vi "Initialization.vi"(8 "error in":errorcluster, 9 "UI Refs":T1, 10 "user event":T2, 11 "XY Plotter":refnum<class "XY Plotter.lvclass">) -> (0 "error out":errorcluster, 3 "XY Plotter out":refnum<class "XY Plotter.lvclass">)   [LabVIEW 2025, in "XY Plotter.lvlib" / "XY Plotter.lvclass"]
uses:
  XY Plotter.lvclass
  Users/Public/Documents/Sandia National Labs/TSS Plugin/CEF.lvlibp/Node/UserEventRef.ctl
  XY Plotter.lvclass/XY Plotter.ctl
  XY Plotter configuration/XY Plotter configuration.lvclass/XY Plotter configuration.ctl
  XY Plotter configuration/Read XY Plotter.vi
  XY Plotter configuration/XY Plotter configuration.lvclass
  Users/Public/Documents/Sandia National Labs/TSS Plugin/CEF.lvlibp/Node/CEF_Node.lvclass
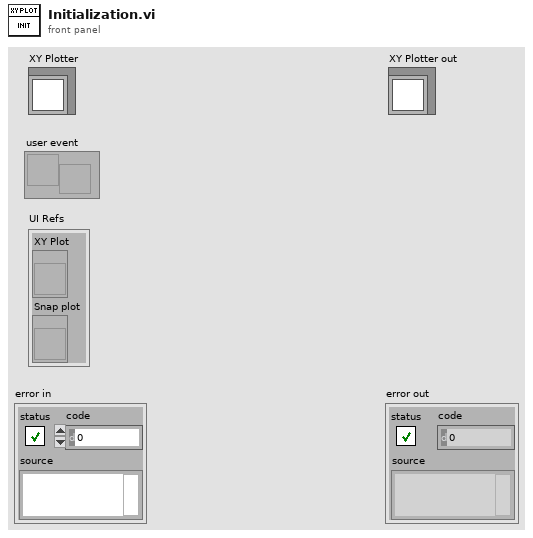
[diagram p1: front panel]
types:
  T1 = cluster{"XY Plot":refnum<vi>, "Snap plot":refnum<vi>}
  T2 = typedef "CEF.lvlibp/CEF_Node.lvclass/UserEventRef.ctl" = refnum<user-event>
  T3 = typedef "XY Plotter.lvlib/XY Plotter configuration.lvclass/XY Plotter.ctl" = cluster{"Data Rate":i32, "Y-Scales":cluster{"Label":string, "Max":dbl, "Min":dbl, "Unit":enum16{"---", "V", "mA", "sec", "dB", "deg", "in/s", "in", "lbf", "Hz", "psi", "gpm"}, "Visible":bool}[], "Note":string, "History Length":i32, "DataLog Path":path, "Plot type":bool, "X-Scales":cluster{"Label":string, "Max":dbl, "Min":dbl, "Unit":enum16{"---", "V", "mA", "sec", "dB", "deg", "in/s", "in", "lbf", "Hz", "psi", "gpm"}, "Visible":bool}[], "Plot List":cluster{"Plot Name":string, "X Scale Index":u32, "Y Scale Index":u32, "Visible":bool}[]}
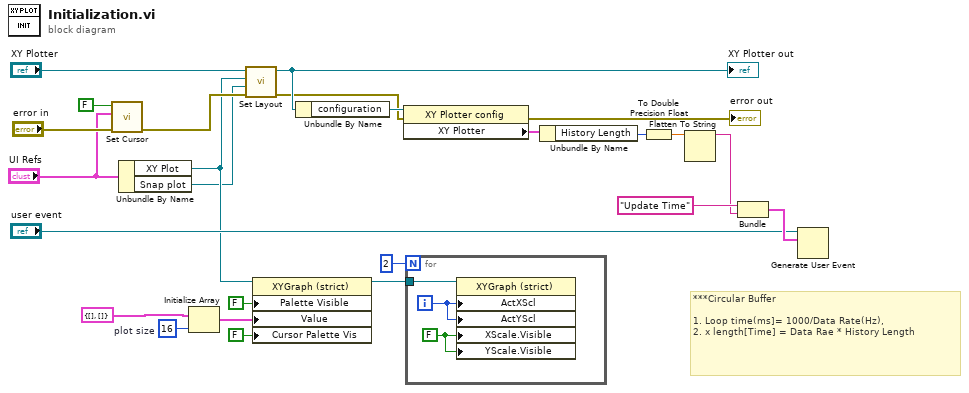
[diagram p0: block diagram]
diagram:
  w22 = 16  # plot size
  # "***Circular Buffer \n\n1. Loop time(ms]= 1000/Data Rate(Hz),\n2. x length[Time] = Data Rae * History Length"
  n1 = call "Set Cursor.vi"("error in (no error)"="error in", "UI Refs"="UI Refs", "Visible(F)"=FALSE) -> ("error out"=w8:errorcluster)  [unwired: 8 in]
  n2 = Unbundle By Name("UI Refs") -> ("XY Plot"=w2:refnum<vi>, "Snap plot"=w1:refnum<vi>)
  n3 = Initialize Array(cluster{"X":dbl[], "Y":dbl[]} {"X"=[], "Y"=[]} ("Spectrum"), w22) -> (w20:cluster{"X":dbl[], "Y":dbl[]}[])
  n4 = call "Set Layout.vi"("error in (no error)"=w8, "Snap plot"=w1, "XY Plot"=w2, "XY Plotter"="XY Plotter") -> ("error out"=w5:errorcluster, "XY Plotter out"=w6:refnum<class "XY Plotter.lvclass">)  [unwired: 6 in]
  "XY Plotter out" <- w6
  n5 = property class="XYGraph (strict)"(reference=w2, "Palette Visible"=FALSE ("Palette:Visible"), "Value"=w20, "Cursor Palette Vis"=FALSE ("Cursor Legend Visible")) -> (reference out=w24:refnum<vi>)  [unwired: 1 in, 1 out]
  n6 = Unbundle By Name(w6) -> ("configuration"=w17:refnum<class "XY Plotter configuration.lvclass">)
  n7 = property class="XY Plotter config"(reference=w17, error in=w5) -> (error out=→"error out":errorcluster, "XY Plotter"=w16:T3)  [unwired: 1 out]
  n8 = for {
    N: 2 -> [_]
    tunnel: w24 -> [w26]
    i -> [w28]
    w27 = FALSE ("X Scale.Visible")
    n9 = property class="XYGraph (strict)"(reference=w26, "ActXScl"=w28, "ActYScl"=w28, "XScale.Visible"=w27, "YScale.Visible"=w27) -> ()  [unwired: 1 in, 2 out]
  }
  n10 = Unbundle By Name(w16) -> ("History Length"=w12:i32)
  n11 = To Double Precision Float(number=w12) -> (double precision float=w11:dbl)
  n12 = Flatten To String(anything=w11) -> (data string=w14:string)  [unwired: 3 in, 2 out]
  n13 = Bundle("message"="Update Time", "data string"=w14) -> (w13:cluster{"message":string, "data string":string})  [unwired: 1 in]
  n14 = Generate User Event(user event="user event", event data cluster=w13) -> ()  [unwired: 2 in, 2 out]
